vi "DO seq_event.vi"(0 "Channel Names":string[](array[string])=["DO00", "DO01", "DO02", "DO03", "DO04", "DO05", "DO06", "DO07", "DO08", "DO09", "DO10", "DO11", "DO12", "DO13", "DO14", "DO15", "DO16", "DO17", "DO18", "DO19", "DO20", "DO21", "DO22", "DO23", "DO24", "DO25", "DO26", "DO27", "DO28", "DO29", "DO30", "DO31", "DO32", "DO33", "DO34", "DO35", "DO36", "DO37", "DO38", "DO39", "DO40", "DO41", "DO42", "DO43", "DO44", "DO45", "DO46", "DO47", "DO48", "DO49", "DO50", "DO51", "DO52", "DO53", "DO54", "DO55", "DO56", "DO57", "DO58", "DO59", "DO60", "DO61", "DO62", "DO63"], 5 "Sequence Table":string[][](array[string])=[["DO01", "1", "5"], ["DO63", "3", "8"]]) -> (4 "DO Output":bool[](array[boolean]), 6 "Time (s)":dbl)   [LabVIEW 2026]
doc: "시퀀스 테이블 기반 DO 출력 시험 VI.\n[시험 시작] 시퀀스 테이블 1열의 채널 이름을 Channel Names 배열에서 검색해 인덱스를 구하고(0부터 시작, DO01=1), 2열 On Time / 3열 Off Time(초)을 숫자로 변환한다. DO Output을 모두 OFF로, Time을 0으로 초기화하고 카운트를 시작한다.\n[실행 중] 50 ms마다 경과 시간 Time(s)을 갱신하고, 각 행의 채널을 On Time <= Time < Off Time 동안 ON, 그 밖에는 OFF로 출력한다.\n[자동 정지] Time이 시퀀스 테이블의 가장 큰 Off Time에 도달하면(>=) 시험을 정지한다.\n[시험 정지] 버튼을 누르면 중간에 정지한다(출력 상태는 유지). 다시 시작하면 출력과 시간이 초기화된다.\n창을 닫으면 VI가 종료된다. 같은 채널이 여러 행에 있으면 아래쪽 행의 판정이 우선한다."
panel:
  in  "Stop":bool
  in  "Start":bool
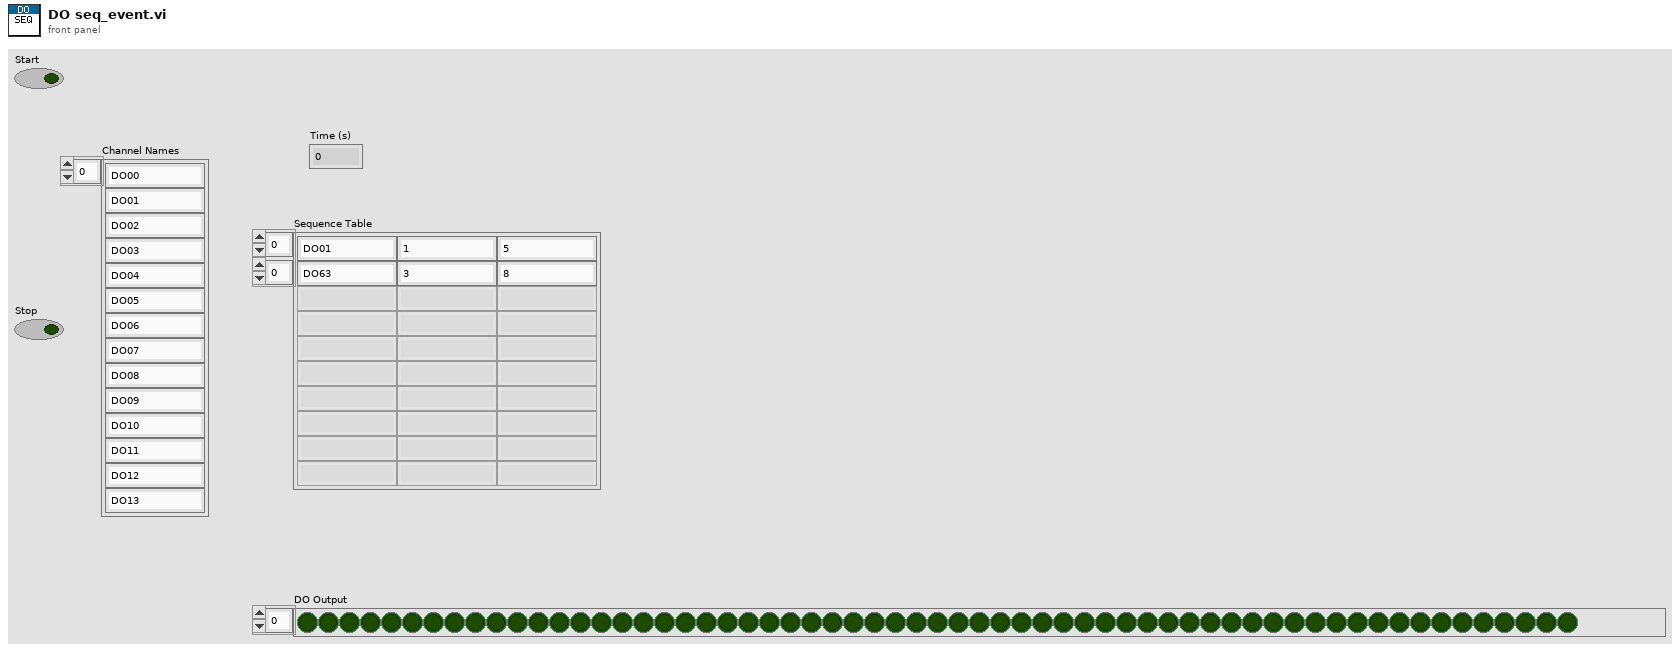
[diagram p1: front panel]
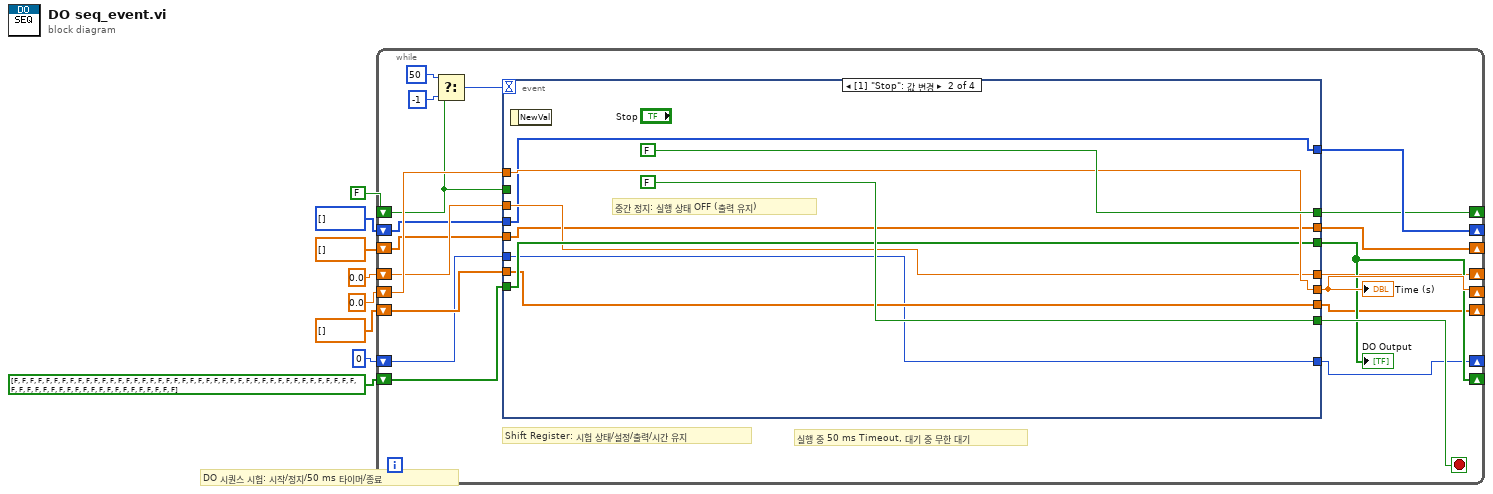
[diagram p0: block diagram]
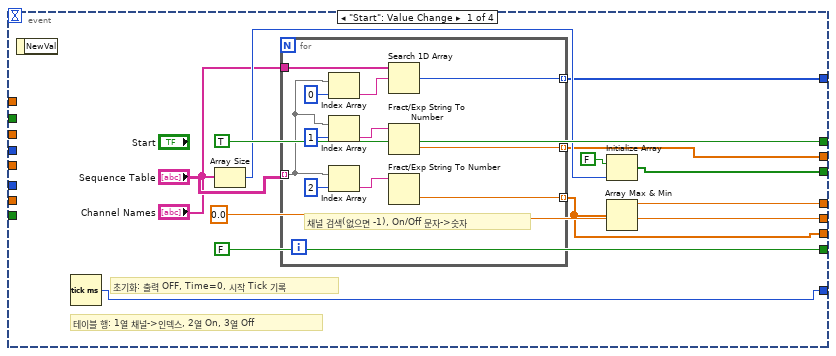
[diagram p2: hidden frame]
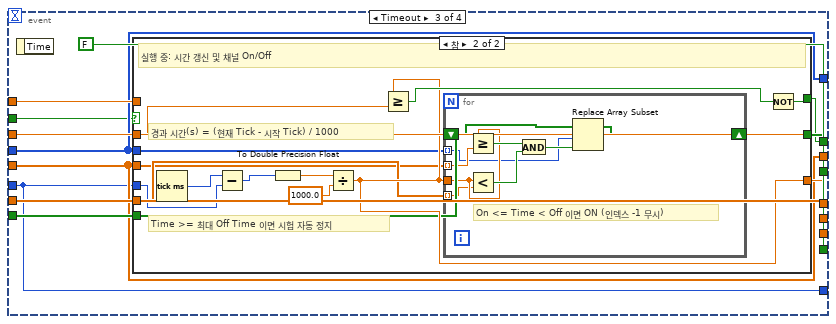
[diagram p3: hidden frame]
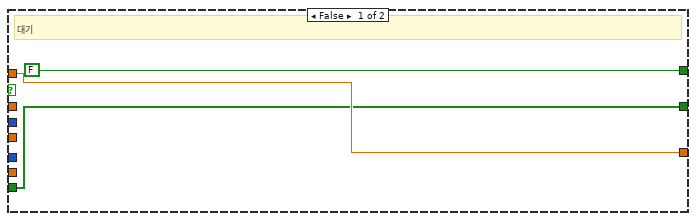
[diagram p4: hidden frame]
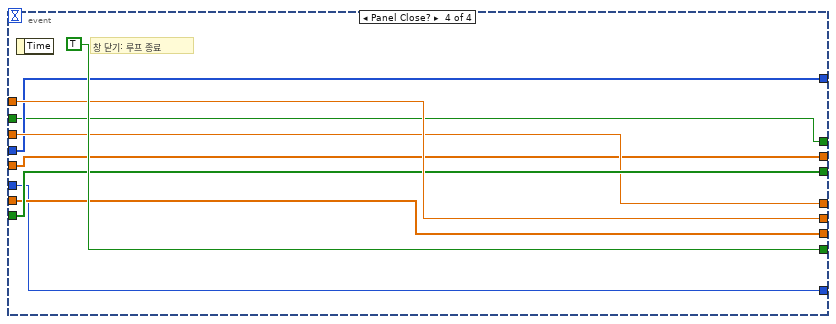
[diagram p5: hidden frame]
diagram:
  # "DO 시퀀스 시험: 시작/정지/50 ms 타이머/종료"
  n1 = while {
    shift-right: [w20] -> _
    shift-left: FALSE -> [w12]
    shift-right: [w21] -> _
    shift-left: u32 0 -> [w13]
    shift-right: [w22] -> _
    shift-left: i32[] [] -> [w14]
    shift-right: [w23] -> _
    shift-left: dbl[] [] -> [w15]
    shift-right: [w24] -> _
    shift-left: dbl[] [] -> [w16]
    shift-right: [w25] -> _
    shift-left: 0.0 -> [w17]
    shift-right: [w26] -> _
    shift-left: bool[] [FALSE, FALSE, FALSE, FALSE, FALSE, FALSE, FALSE, FALSE, FALSE, FALSE, FALSE, FALSE, FALSE, FALSE, FALSE, FALSE, FALSE, FALSE, FALSE, FALSE, FALSE, FALSE, FALSE, FALSE, FALSE, FALSE, FALSE, FALSE, FALSE, FALSE, FALSE, FALSE, FALSE, FALSE, FALSE, FALSE, FALSE, FALSE, FALSE, FALSE, FALSE, FALSE, FALSE, FALSE, FALSE, FALSE, FALSE, FALSE, FALSE, FALSE, FALSE, FALSE, FALSE, FALSE, FALSE, FALSE, FALSE, FALSE, FALSE, FALSE, FALSE, FALSE, FALSE, FALSE] -> [w18]
    shift-right: [w27] -> _
    shift-left: 0.0 -> [w19]
    stop <- w28 stop-if-true
    # "실행 중 50 ms Timeout, 대기 중 무한 대기"
    # "Shift Register: 시험 상태/설정/출력/시간 유지"
    n2 = Select(t=50, s=w12, f=-1) -> (s? t:f=w11:i32)
    n3 = event shown="[1] \"Stop\": 값 변경" {
      selector: _ -> [_ _ _ _]
      dyn-events: _ -> [_ _ _ _]
      timeout: w11 -> [_ _ _ _]
      tunnel: [TRUE FALSE w70 w100] -> w20
      tunnel: [0.0 w59 w72 w107] -> w27
      tunnel: [FALSE FALSE FALSE TRUE] -> w28
      tunnel: w12 -> [_ _ w62 w100]
      tunnel: w13 -> [_ w53 w63 w101]
      tunnel: w14 -> [_ w54 w64 w102]
      tunnel: w15 -> [_ w55 w65 w103]
      tunnel: w16 -> [_ w56 w66 w104]
      tunnel: w17 -> [_ w57 w67 w105]
      tunnel: w18 -> [_ w58 w68 w106]
      tunnel: w19 -> [_ w59 w69 w107]
      tunnel: [w38 w53 w63 w101] -> w21
      tunnel: [w37 w58 w71 w106] -> w26
      tunnel: [w31 w54 w64 w102] -> w22
      tunnel: [w32 w55 w65 w103] -> w23
      tunnel: [w33 w56 w66 w104] -> w24
      tunnel: [w34 w57 w67 w105] -> w25
      event "Start": Value Change {
        # "초기화: 출력 OFF, Time=0, 시작 Tick 기록"
        # "테이블 행: 1열 채널->인덱스, 2열 On, 3열 Off"
        n4 = event-data() -> ()  [unwired: 1 in, 1 out]
        n5 = Tick Count (ms)() -> (millisecond timer value=w38:u32)
        n6 = Array Size(array="Channel Names") -> (size(s)=w35:i32)
        n7 = for {
          tunnel: "Sequence Table" -> [w42] mode=indexing
          tunnel: "Channel Names" -> [w43]
          tunnel: [w50] -> w31 mode=indexing
          tunnel: [w51] -> w32 mode=indexing
          tunnel: [w52] -> w33 mode=indexing
          # "채널 검색(없으면 -1), On/Off 문자->숫자"
          n8 = Index Array(array=w42, index=0) -> (element=w47:string)
          n9 = Index Array(array=w42, index=1) -> (element=w48:string)
          n10 = Index Array(array=w42, index=2) -> (element=w49:string)
          n11 = Search 1D Array(1D array=w43, element=w47) -> (index of element=w50:i32)  [unwired: 1 in]
          n12 = Fract/Exp String To Number(string=w48) -> (number=w51:dbl)  [unwired: 3 in, 1 out]
          n13 = Fract/Exp String To Number(string=w49) -> (number=w52:dbl)  [unwired: 3 in, 1 out]
        }
        n14 = Initialize Array(FALSE, w35) -> (w37:bool[])
        n15 = Array Max & Min(array=w33) -> (max value=w34:dbl)  [unwired: 3 out]
      }
      event "Stop": Value Change {
        # "중간 정지: 실행 상태 OFF (출력 유지)"
        n16 = event-data() -> ()  [unwired: 1 in, 1 out]
      }
      event Timeout {
        n17 = event-data() -> ()  [unwired: 1 in, 1 out]
        n18 = case shown="참" w62 {
          tunnel: w63 -> [_ w77]
          tunnel: w64 -> [_ w78]
          tunnel: w65 -> [_ w79]
          tunnel: w66 -> [_ w80]
          tunnel: w67 -> [_ w81]
          tunnel: w68 -> [w74 w82]
          tunnel: w69 -> [w75 _]
          tunnel: [w74 w88] -> w71
          tunnel: [w75 w87] -> w72
          tunnel: [FALSE w90] -> w70
          frame False {
            # "대기"
          }
          frame True {
            # "Time >= 최대 Off Time 이면 시험 자동 정지"
            # "경과 시간(s) = (현재 Tick - 시작 Tick) / 1000"
            # "실행 중: 시간 갱신 및 채널 On/Off"
            n19 = Tick Count (ms)() -> (millisecond timer value=w83:u32)
            n20 = Subtract(x=w83, y=w77) -> (x-y=w84:u32)
            n21 = To Double Precision Float(number=w84) -> (double precision float=w85:dbl)
            n22 = Divide(x=w85, y=1000.0) -> (x/y=w87:dbl)
            n23 = Greater Or Equal?(x=w87, y=w81) -> (x >= y?=w89:bool)
            n24 = for {
              tunnel: w78 -> [w91] mode=indexing
              tunnel: w79 -> [w92] mode=indexing
              tunnel: w80 -> [w93] mode=indexing
              shift-right: [w98] -> w88
              shift-left: w82 -> [w99]
              tunnel: w87 -> [w94]
              # "On <= Time < Off 이면 ON (인덱스 -1 무시)"
              n25 = Greater Or Equal?(x=w94, y=w92) -> (x >= y?=w95:bool)
              n26 = Less?(x=w94, y=w93) -> (x < y?=w96:bool)
              n27 = And(x=w95, y=w96) -> (x .and. y?=w97:bool)
              n28 = Replace Array Subset(array=w99, new element=w97, index=w91) -> (w98:bool[])
            }
            n29 = Not(x=w89) -> (.not. x?=w90:bool)
          }
        }
      }
      event Panel Close? {
        # "창 닫기: 루프 종료"
        n30 = event-data() -> ()  [unwired: 2 in, 1 out]
        n31 = event-data() -> ()  [unwired: 1 in, 1 out]
      }
    }
    "DO Output" <- w26
    "Time (s)" <- w27
  }
